vi "Change Message Data.vi"(8 "error in":errorcluster, 10 "Message Data":variant, 11 "Helper Loop":refnum<class "Helper Loop.lvclass">) -> (0 "error out":errorcluster, 3 "Helper Loop Out":refnum<class "Helper Loop.lvclass">)   [LabVIEW 2020, in "Helper Loop.lvclass"]
doc: "周期的に送るメッセージデータを変更します。\n変更すると、それまで経過した時間がリセットされます。"
uses:
  Helper Loop.lvclass
  Helper Loop.lvclass/Helper Loop.ctl
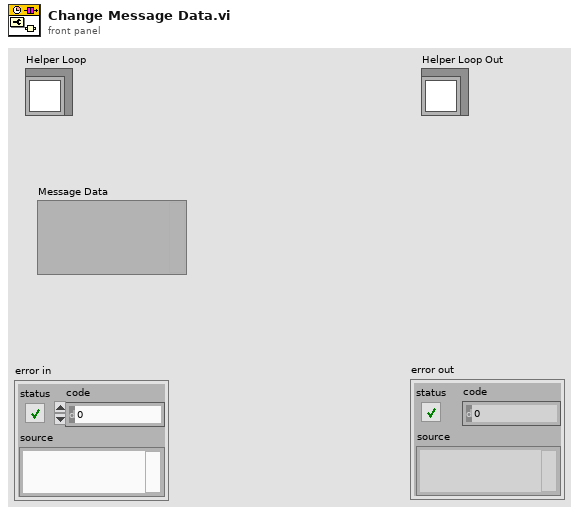
[diagram p1: front panel]
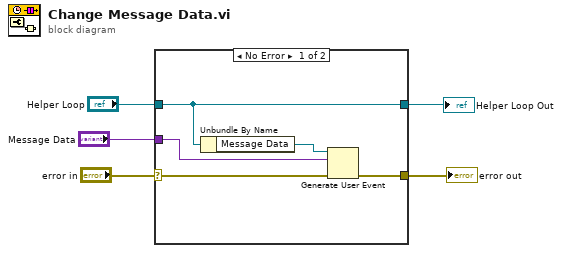
[diagram p0: block diagram]
diagram:
  n1 = case shown="No Error" "error in" {
    selector: "error in" -> [w8 w12]
    tunnel: [w7 w12] -> w4
    tunnel: "Helper Loop" -> [w10 w11]
    tunnel: [w10 w11] -> w2
    tunnel: "Message Data" -> [w6 _]
    frame No Error {
      n2 = Unbundle By Name(w10) -> ("Message Data"=w9:refnum<user-event>)
      n3 = Generate User Event(user event=w9, event data cluster=w6, error in=w8) -> (error out=w7:errorcluster)  [unwired: 1 in, 1 out]
    }
    frame Error {
    }
  }
  "error out" <- w4
  "Helper Loop Out" <- w2
